vi "DropVI_SimpleClientPublisher.vi"() -> ()   [LabVIEW 2013, in "MQTT Client.lvlib"]
uses:
  MQTT Client.lvlib
  Client class/Client.lvclass/Client.ctl
  <vilib>/LabVIEW Open Source Project/MQTT Connection/MQTT_Base/Base Class/MQTT_Base.lvclass/MQTT_Base.ctl
  <vilib>/LabVIEW Open Source Project/MQTT Control Packets/Control Packets/PUBLISH/PUBLISH.lvclass
  Client class/Client.lvclass
  <vilib>/LabVIEW Open Source Project/MQTT Connection/MQTT_Base/Base Class/MQTT_Base.lvclass
  <vilib>/LabVIEW Open Source Project/Connection/Connection/Connection.lvclass
  <vilib>/LabVIEW Open Source Project/Connection/Connection.TCP/Connection.TCP.lvclass
  <vilib>/LabVIEW Open Source Project/Connection/Connection.LocalQueue/Connection.LocalQueue.lvclass
panel:
  out "last error":errorcluster
  in  "Connection":bool
  out "Waveform Chart":dbl(graph)
  out "Published":bool
  in  "Stop Client":bool
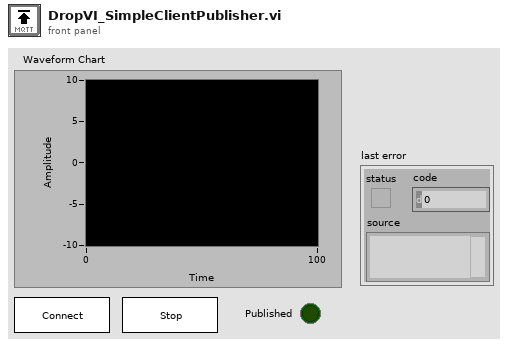
[diagram p1: front panel]
types:
  T1 = typedef "MQTT Client.lvlib/Client.lvclass/Public Events -- cluster.ctl" = cluster{"Connection Status":refnum<user-event>, "Connected":refnum<user-event>, "Application Message":refnum<user-event>}
  T2 = typedef "MQTT Base.lvlib/MQTT_Base.lvclass/Public Events -- cluster.ctl" = cluster{"Stop Event":refnum<user-event>, "Error Event":refnum<user-event>, "Inbound Message":refnum<user-event>}
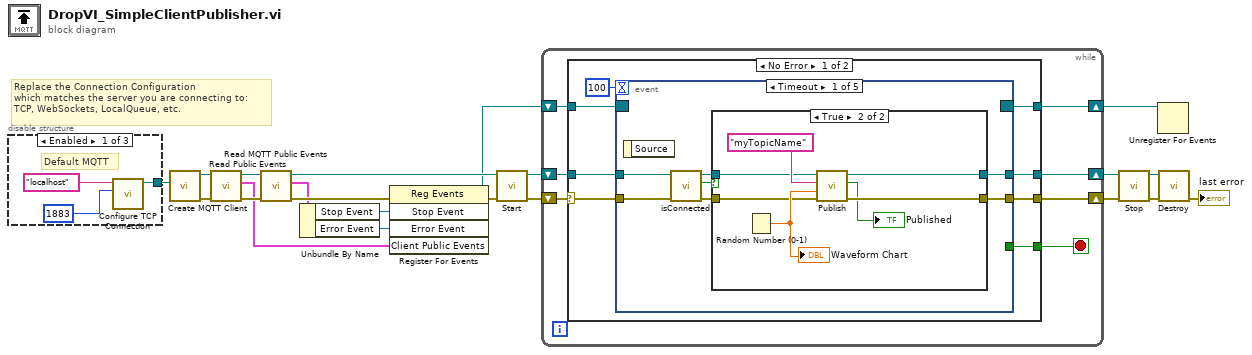
[diagram p0: block diagram]
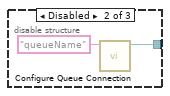
[diagram p2: hidden frame]
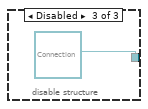
[diagram p3: hidden frame]
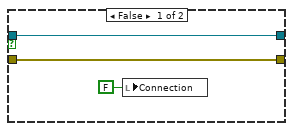
[diagram p4: hidden frame]
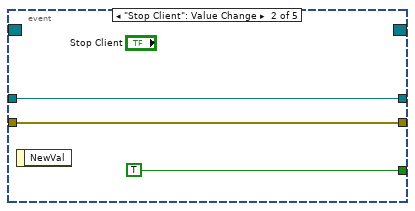
[diagram p5: hidden frame]
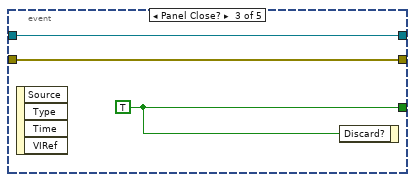
[diagram p6: hidden frame]
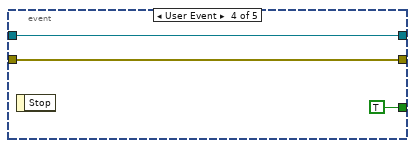
[diagram p7: hidden frame]
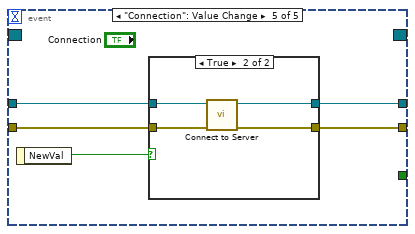
[diagram p8: hidden frame]
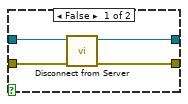
[diagram p9: hidden frame]
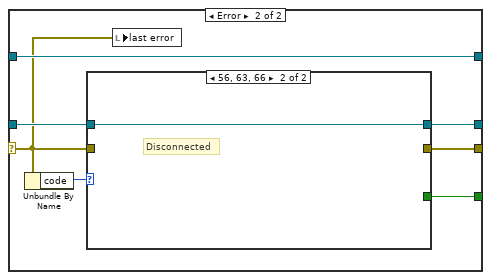
[diagram p10: hidden frame]
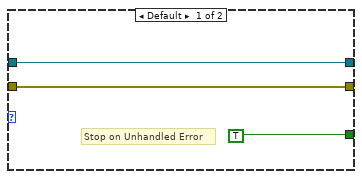
[diagram p11: hidden frame]
diagram:
  # "Replace the Connection Configuration\nwhich matches the server you are connecting to:\nTCP, WebSockets, LocalQueue, etc."
  n1 = disable-structure shown="Enabled" {
    disable-tunnel: [w23 w26 refnum<class "Connection.lvclass"> refnum ("Connection Configuration")] -> w1
    frame Enabled {
      # "Default MQTT"
      n2 = call <vilib>:"Configure TCP Connection.vi"("remote port (80)"=u16 1883, "address (localhost)"="localhost") -> ("Connection.TCP"=w23:refnum<class "Connection.TCP.lvclass">)  [unwired: 8 in, 1 out]
    }
    frame Disabled {
      n3 = call <vilib>:"Configure Queue Connection.vi"("Queue Name"="queueName") -> ("Connection.LocalQueue"=w26:refnum<class "Connection.LocalQueue.lvclass">)  [unwired: 9 in, 1 out]
    }
    frame Disabled {
    }
  }
  n4 = call "Create MQTT Client.vi"("Connection Configuration"=w1) -> ("error out"=w19:errorcluster, "Client out"=w21:refnum<class "Client.lvclass">)  [unwired: 9 in]
  n5 = call "Read Public Events.vi"("error in (no error)"=w19, "Client in"=w21) -> ("error out"=w18:errorcluster, "Client Public Events"=w16:T1, "Client out"=w20:refnum<class "Client.lvclass">)  [unwired: 7 in]
  n6 = call <vilib>:"Read MQTT Public Events.vi"("error in (no error)"=w18, "MQTT_Base in"=w20) -> ("error out"=w17:errorcluster, "MQTT Public Events"=w9:T2, "MQTT_Base out"=w14:refnum<class "Client.lvclass">)  [unwired: 7 in]
  n7 = Unbundle By Name(w9) -> ("Stop Event"=w11:refnum<user-event>, "Error Event"=w10:refnum<user-event>)
  n8 = register-events(error in=w17, w11, w10, w16) -> (reference out=w13:refnum<event-registration>, error out=w15:errorcluster)  [unwired: 1 in]
  n9 = call <vilib>:"Start.vi"("error in (no error)"=w15, "MQTT_Base in"=w14) -> ("error out"=w3:errorcluster, "MQTT_Base out"=w4:refnum<class "Client.lvclass">)  [unwired: 7 in, 1 out]
  n10 = while {
    shift-right: [w33] -> w12
    shift-left: w13 -> [w34]
    shift-right: [w30] -> w7
    shift-left: w4 -> [w31]
    shift-right: [w32] -> w5
    shift-left: w3 -> [w28]
    stop <- w29 stop-if-true
    n11 = case shown="No Error" w28 {
      selector: w28 -> [w35 w82]
      tunnel: w34 -> [w42 w88]
      tunnel: [w41 w88] -> w33
      tunnel: [w40 w84] -> w32
      tunnel: w31 -> [w38 w86]
      tunnel: [w37 w85] -> w30
      tunnel: [w36 w83] -> w29
      frame No Error {
        n12 = event shown="[0] Timeout" {
          selector: w42 -> [_ _ _ _ _]
          dyn-events: [_ _ _ _ _] -> w41
          timeout: 100 -> [_ _ _ _ _]
          tunnel: w35 -> [w45 w61 w63 w68 w69]
          tunnel: [w48 w61 w63 w68 w70] -> w40
          tunnel: [_ TRUE w65 TRUE _] -> w36
          tunnel: w38 -> [w47 w62 w64 w66 w73]
          tunnel: [w49 w62 w64 w66 w71] -> w37
          event Timeout {
            n13 = event-data() -> ()  [unwired: 1 in, 1 out]
            n14 = call "isConnected.vi"("error in (no error)"=w45, "Client in"=w47) -> ("error out"=w44:errorcluster, "connected"=w43:bool, "Client out"=w46:refnum<class "Client.lvclass">)  [unwired: 7 in]
            n15 = case shown="True" w43 {
              tunnel: [w52 w58] -> w49
              tunnel: [w51 w57] -> w48
              tunnel: w46 -> [w52 w54]
              tunnel: w44 -> [w51 w53]
              frame False {
                n16 = local write "Connection"(FALSE ("Connection")) -> ()
              }
              frame True {
                n17 = Random Number (0-1)() -> (number: 0 to 1=w55:dbl)
                "Waveform Chart" <- w55
                n18 = call "Publish.vi"("error in (no error)"=w53, "Payload"=w55, "Topic Name (empty: Payload name)"="myTopicName", "Client in"=w54) -> ("error out"=w57:errorcluster, "Published"=→"Published":bool, "Client out"=w58:refnum<class "Client.lvclass">)  [unwired: 5 in]
              }
            }
          }
          event "Stop Client": Value Change {
            n19 = event-data() -> ()  [unwired: 1 in, 1 out]
          }
          event Panel Close? {
            w65 = TRUE
            n20 = event-data() -> ()  [unwired: 1 in, 4 out]
            n21 = event-data("Discard?"=w65) -> ()  [unwired: 1 in, 1 out]
          }
          event User Event {
            n22 = event-data() -> ()  [unwired: 1 in, 1 out]
          }
          event "Connection": Value Change {
            n23 = event-data() -> ("NewVal"=w72:bool)  [unwired: 1 in]
            n24 = case shown="True" w72 {
              tunnel: w73 -> [w77 w81]
              tunnel: [w76 w78] -> w71
              tunnel: [w75 w79] -> w70
              tunnel: w69 -> [w74 w80]
              frame False {
                n25 = call "Disconnect from Server.vi"("error in (no error)"=w74, "Client in"=w77) -> ("error out"=w75:errorcluster, "Client out"=w76:refnum<class "Client.lvclass">)  [unwired: 7 in, 1 out]
              }
              frame True {
                n26 = call "Connect to Server.vi"("error in (no error)"=w80, "Client in"=w81) -> ("error out"=w79:errorcluster, "Client out"=w78:refnum<class "Client.lvclass">)  [unwired: 6 in, 2 out]
              }
            }
          }
        }
      }
      frame Error {
        n27 = Unbundle By Name(w82) -> ("code"=w87:i32)
        n28 = case shown="56, 63, 66" w87 {
          tunnel: w86 -> [w91 w92]
          tunnel: [w91 w92] -> w85
          tunnel: w82 -> [w90 _]
          tunnel: [w90 _] -> w84
          tunnel: [TRUE _] -> w83
          frame Default {
            # "Stop on Unhandled Error"
          }
          frame 56, 63, 66 {
            # "Disconnected"
          }
        }
        n29 = local write "last error"(w82) -> ()
      }
    }
  }
  n30 = call <vilib>:"Stop.vi"("error in (no error)"=w5, "MQTT_Base in"=w7) -> ("error out"=w6:errorcluster, "MQTT_Base out"=w8:refnum<class "Client.lvclass">)  [unwired: 7 in, 1 out]
  n31 = Unregister For Events(event registration refnum=w12) -> ()  [unwired: 1 in, 1 out]
  n32 = call <vilib>:"Destroy.vi"("error in (no error)"=w6, "MQTT_Base in"=w8) -> ("error out"=→"last error":errorcluster)  [unwired: 8 in, 1 out]
